vi "Init Data Handling.vi"(4 "Channels per Group":cluster{cluster{"Index":i32, "Name":string}[]}[](array[cluster]), 6 "Groups":string[](array[string]), 8 "error in (no error)":errorcluster, 9 "Channels":string[](array[string]), 10 "Buffer Size":i32, 11 "LocalGraphBuffer in":refnum<class "LocalGraphBuffer.lvclass">) -> (0 "error out":errorcluster, 3 "LocalGraphBuffer out":refnum<class "LocalGraphBuffer.lvclass">)   [LabVIEW 2020, in "VolatusGUIElements.lvlib" / "LocalGraphBuffer.lvclass"]
uses:
  LocalGraphBuffer.lvclass
  Plot.ctl
  lv-vecto/Vecto/Subscribed Data.ctl
  LocalGraphBuffer.lvclass/LocalGraphBuffer.ctl
  <vilib>/Utility/miscctls.llb/LVMapReplaceAction.ctl
  lv-vecto/Vecto/Vecto.lvlib
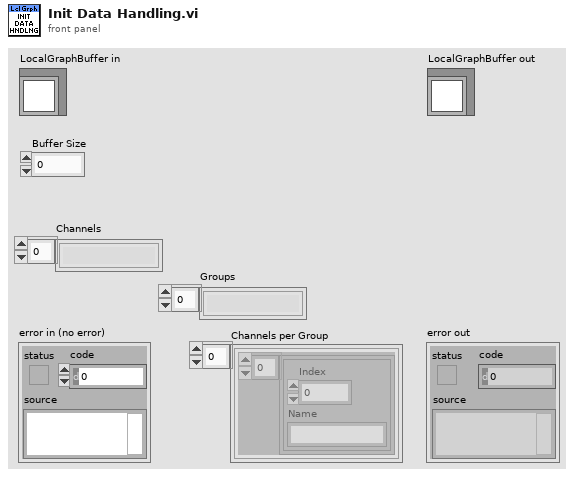
[diagram p1: front panel]
types:
  T1 = typedef "Vecto.lvlib/Subscribed Data.ctl" = cluster{"Group":string, "Timestamp":dbl, "Data":dbl[], "Received Time":dbl}
  T2 = typedef "VolatusGUIElements.lvlib/LocalGraphBuffer.lvclass/Plot.ctl" = cluster{"Data Q":refnum<queue>, "Time Q":refnum<queue>, "Group":string, "Channel Index":i32}
  T3 = typedef "VolatusGUIElements.lvlib/LocalGraphBuffer.lvclass/Group Sub.ctl" = cluster{"Plot Indices":i32[]}
  T4 = typedef "LVMapReplaceAction.ctl" = enum32{"Modify Entry only if found", "Add or Modify Entry", "Delete Entry"}
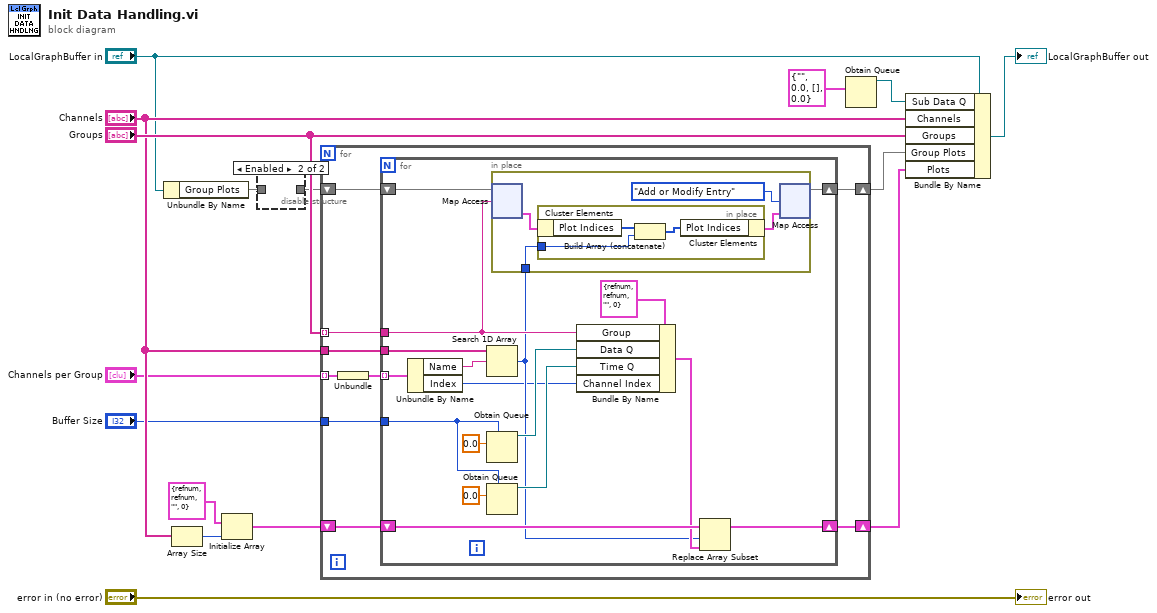
[diagram p0: block diagram]
diagram:
  n1 = Unbundle By Name("LocalGraphBuffer in") -> ("Group Plots"=w6:map{string, T3})
  n2 = Array Size(array="Channels") -> (size(s)=w13:i32)
  n3 = Initialize Array(T2 {"Data Q"=refnum, "Time Q"=refnum, "Group"="", "Channel Index"=0} ("Plot"), w13) -> (w11:T2[])
  n4 = disable-structure shown="Enabled" {
    disable-tunnel: [w17 _] -> w7
    disable-tunnel: w6 -> [w17 _]
    frame Disabled {
    }
    frame Enabled {
    }
  }
  n5 = for {
    tunnel: "Groups" -> [w22] mode=indexing
    tunnel: "Channels per Group" -> [w26] mode=indexing
    shift-right: [w21] -> w9
    shift-left: w11 -> [w23]
    tunnel: "Channels" -> [w25]
    shift-right: [w19] -> w5
    shift-left: w7 -> [w20]
    tunnel: "Buffer Size" -> [w18]
    n6 = Unbundle(w26) -> (w24:cluster{"Index":i32, "Name":string}[])
    n7 = for {
      tunnel: w25 -> [w43]
      tunnel: w24 -> [w29] mode=indexing
      shift-right: [w35] -> w21
      shift-left: w23 -> [w37]
      tunnel: w22 -> [w33]
      shift-right: [w32] -> w19
      shift-left: w20 -> [w34]
      tunnel: w18 -> [w30]
      n8 = Unbundle By Name(w29) -> ("Name"=w28:string, "Index"=w27:i32)
      n9 = Search 1D Array(1D array=w43, element=w28) -> (index of element=w31:i32)  [unwired: 1 in]
      n10 = Obtain Queue(max queue size (-1, unlimited)=w30, element data type=0.0) -> (queue out=w40:refnum<queue>)  [unwired: 3 in, 2 out]
      n11 = Obtain Queue(max queue size (-1, unlimited)=w30, element data type=0.0) -> (queue out=w38:refnum<queue>)  [unwired: 3 in, 2 out]
      n12 = in-place {
        in-place-border: w31 -> [w44]
        n13 = in-place-map #1(w34, w33) -> (w46:T3)  [unwired: 1 in, 1 out]
        n14 = in-place {
          in-place-border: w44 -> [w48]
          n15 = in-place-cluster #2(w46) -> ("Plot Indices"=w50:i32[])
          n16 = Build Array (concatenate)(w50, w48) -> (w49:i32[])
          n17 = in-place-cluster #2("Plot Indices"=w49) -> (w45:T3)
        }
        n18 = in-place-map #1(w45, LVMapReplaceAction."Add or Modify Entry" ("action")) -> (w32:map{string, T3})  [unwired: 2 out]
      }
      n19 = Bundle By Name(cluster=T2 {"Data Q"=refnum, "Time Q"=refnum, "Group"="", "Channel Index"=0} ("Plot"), "Group"=w33, "Data Q"=w40, "Time Q"=w38, "Channel Index"=w27) -> (w36:T2)
      n20 = Replace Array Subset(array=w37, new element=w36, index=w31) -> (w35:T2[])
    }
  }
  n21 = Obtain Queue(element data type=T1 {"Group"="", "Timestamp"=0.0, "Data"=[], "Received Time"=0.0} ("Subscribed Data")) -> (queue out=w2:refnum<queue>)  [unwired: 4 in, 2 out]
  n22 = Bundle By Name(cluster="LocalGraphBuffer in", "Sub Data Q"=w2, "Channels"="Channels", "Groups"="Groups", "Group Plots"=w5, "Plots"=w9) -> (→"LocalGraphBuffer out":refnum<class "LocalGraphBuffer.lvclass">)
  "error out" <- "error in (no error)"
